vi "fake_arduino.vi"() -> ()   [LabVIEW 2026]
panel:
  out "배터리 패킷":string
  out "배터리(V)":dbl
  in  "stop":bool
  out "거리 패킷":string
  out "거리(cm)":i32
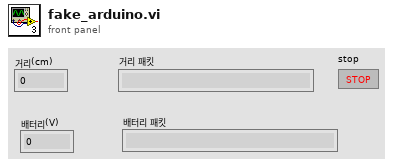
[diagram p1: front panel]
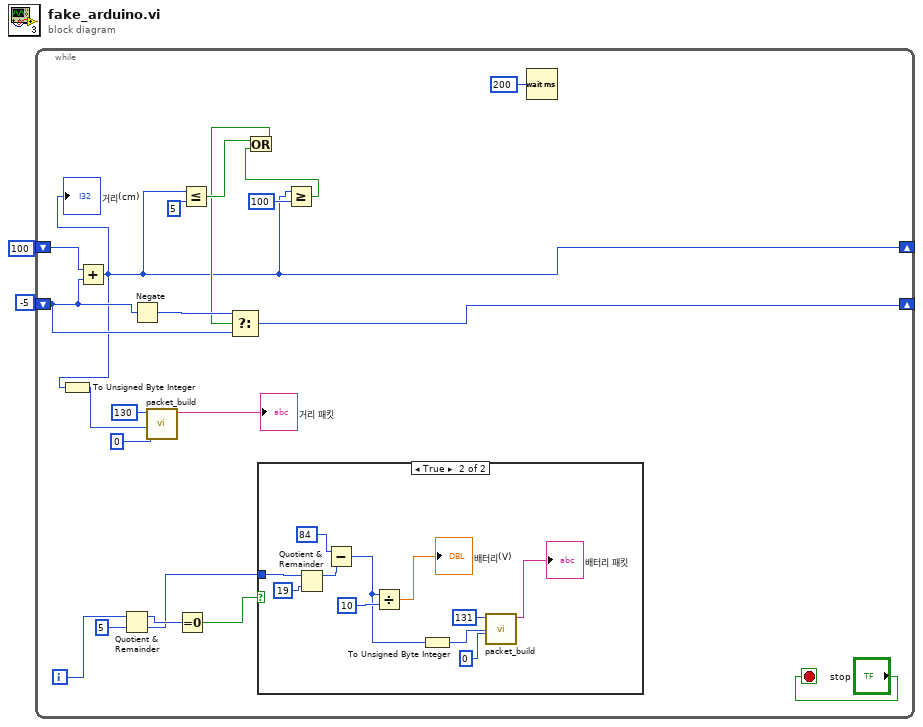
[diagram p0: block diagram]
diagram:
  n1 = while {
    shift-right: [w11] -> _
    shift-left: 100 -> [w22]
    shift-right: [w13] -> _
    shift-left: -5 -> [w14]
    i -> [w8]
    stop <- "stop" stop-if-true
    n2 = Add(x=w22, y=w14) -> (x+y=w11:i32)
    "거리(cm)" <- w11
    n3 = To Unsigned Byte Integer(number=w11) -> (unsigned 8bit integer=w10:u8)
    n4 = Quotient & Remainder(x=w8, y=5) -> (x-y*floor(x/y)=w6:i32, floor(x/y)=w4:i32)
    n5 = Negate(x=w14) -> (-x=w16:i32)
    n6 = call "packet_build.vi"("D2"=u8 0, "D1"=w10, "CMD"=u8 130) -> ("packet"=→"거리 패킷":string)  [unwired: 8 in]
    n7 = Equal To 0?(x=w6) -> (x = 0?=w5:bool)
    n8 = Less Or Equal?(x=w11, y=5) -> (x <= y?=w19:bool)
    n9 = case shown="True" w5 {
      tunnel: w4 -> [_ w34]
      frame False {
      }
      frame True {
        n10 = Quotient & Remainder(x=w34, y=19) -> (x-y*floor(x/y)=w32:i32)  [unwired: 1 out]
        n11 = Subtract(x=84, y=w32) -> (x-y=w27:i32)
        n12 = Divide(x=w27, y=10) -> (x/y=→"배터리(V)":dbl)
        n13 = To Unsigned Byte Integer(number=w27) -> (unsigned 8bit integer=w26:u8)
        n14 = call "packet_build.vi"("D2"=u8 0, "D1"=w26, "CMD"=u8 131) -> ("packet"=→"배터리 패킷":string)  [unwired: 8 in]
      }
    }
    n15 = Greater Or Equal?(x=w11, y=100) -> (x >= y?=w18:bool)
    n16 = Or(x=w19, y=w18) -> (x .or. y?=w15:bool)
    n17 = Select(t=w16, s=w15, f=w14) -> (s? t:f=w13:i32)
    n18 = Wait (ms)(milliseconds to wait=u32 200) -> ()  [unwired: 1 out]
  }
